vi "main battery tester vi22.vi"() -> ()   [LabVIEW 2019]
uses:
  Test_State_Enum.ctl
panel:
  out "system fault":bool
  in  "Start":bool
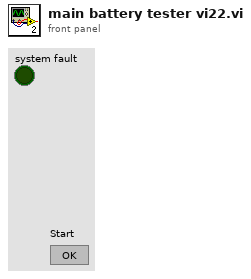
[diagram p1: front panel]
types:
  T1 = enum16{"open", "open or create", "create or replace", "create", "open (read-only)"}
  T2 = typedef "Test_State_Enum.ctl" = enum16{"INIT", "IDLE", "CHARGE _CC", "CHARGE _CV", "REST", "DISCHARGE_DC", "Fault", "Stop"}
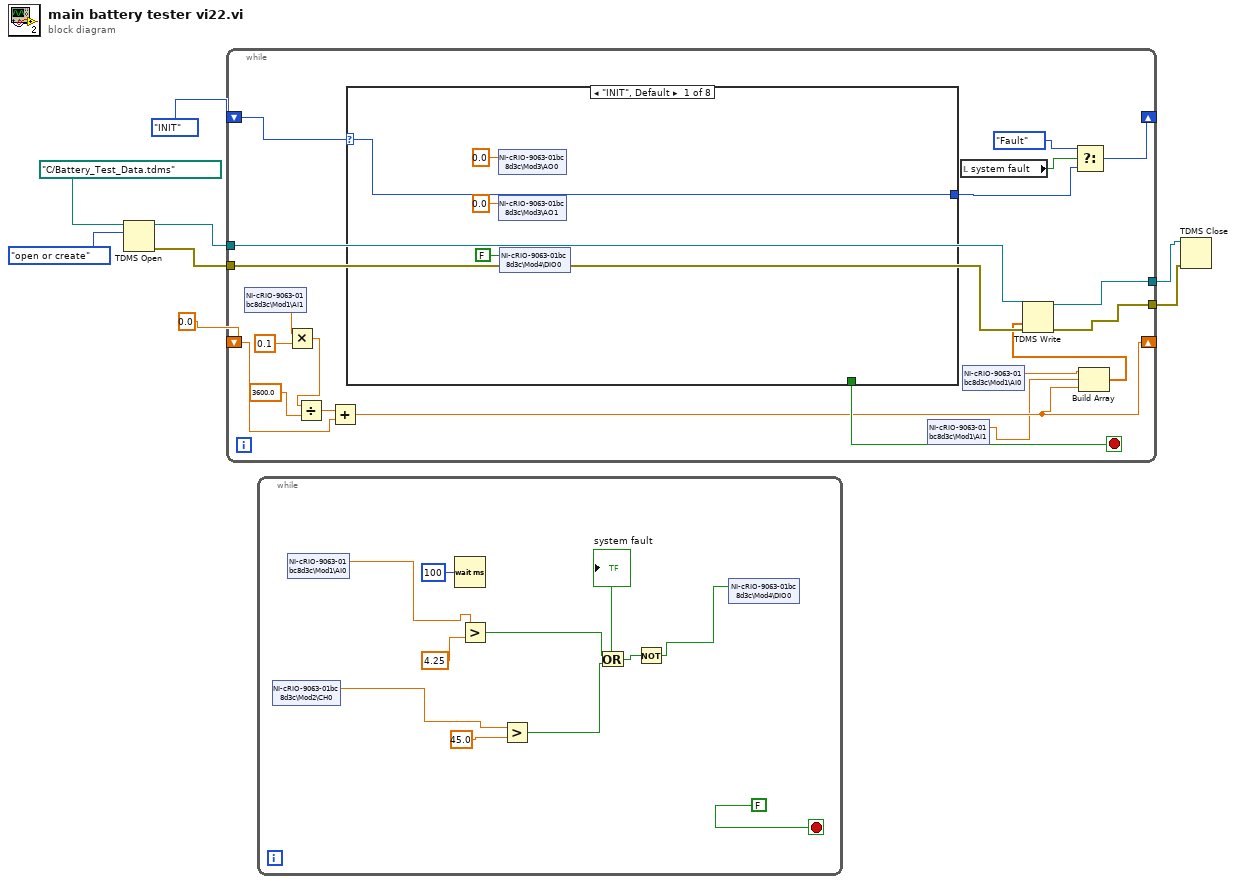
[diagram p0: block diagram]
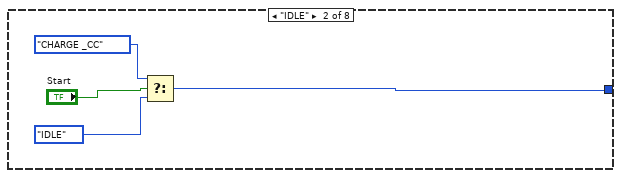
[diagram p2: hidden frame]
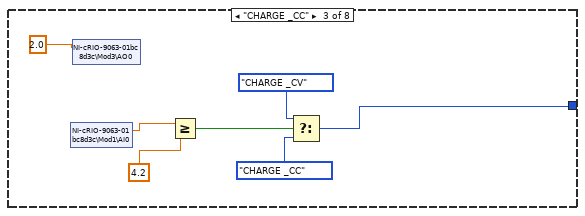
[diagram p3: hidden frame]
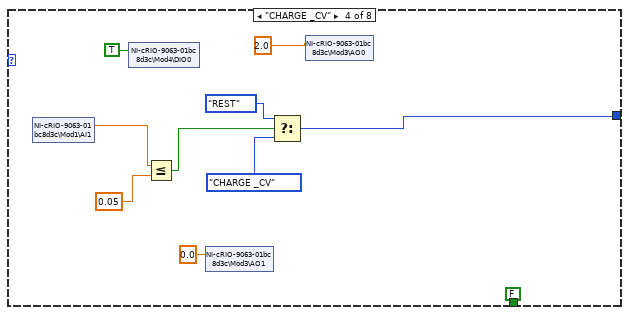
[diagram p4: hidden frame]
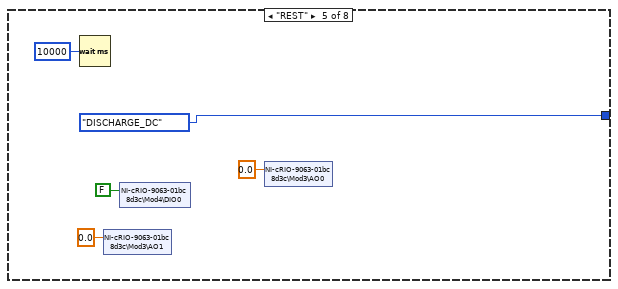
[diagram p5: hidden frame]
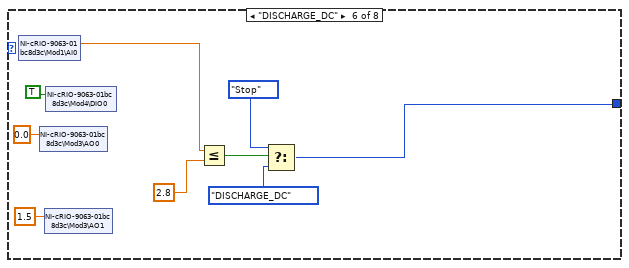
[diagram p6: hidden frame]
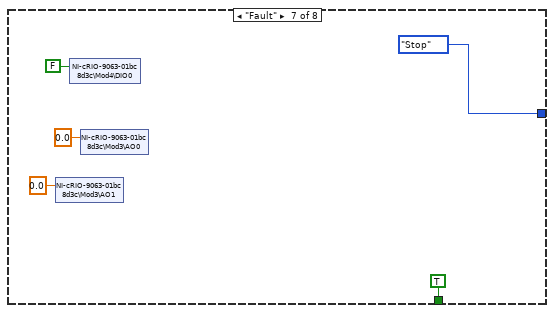
[diagram p7: hidden frame]
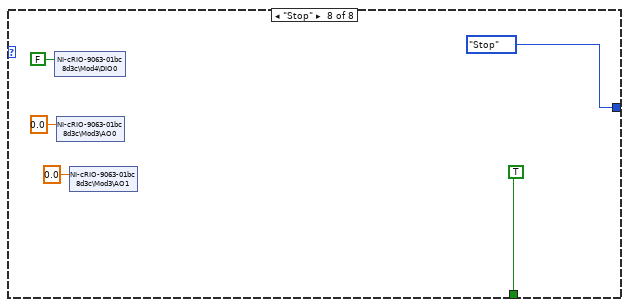
[diagram p8: hidden frame]
diagram:
  n1 = TDMS Open(10:T1."open or create" ("operation (0:open)"), 11:path "C:/Battery_Test_Data.tdms" ("file path")) -> (0:w5:errorcluster, 3:w6:refnum<k34>)  [unwired: 5 in]
  n2 = while {
    shift-right: [w23] -> _
    shift-left: Test_State_Enum."INIT" ("Enum") -> [w28]
    tunnel: w6 -> [w18]
    tunnel: w5 -> [w17]
    shift-right: [w16] -> _
    shift-left: 0.0 -> [w11]
    tunnel: [w15] -> w3
    tunnel: [w14] -> w2
    stop <- w27 stop-if-true
    n3 = shared-variable "NI-cRIO-9063-01bc8d3c\\Mod1\\AI1"() -> (w12:dbl)  [unwired: 1 in, 1 out]
    n4 = Multiply(x=w12, y=0.1) -> (x*y=w21:dbl)
    n5 = Divide(x=w21, y=3600.0) -> (x/y=w19:dbl)
    n6 = Add(x=w19, y=w11) -> (x+y=w16:dbl)
    n7 = case shown="\"INIT\", Default" w28 {
      selector: w28 -> [w29 _ _ _ _ _ _ _]
      tunnel: [w29 w34 w42 w49 Test_State_Enum."DISCHARGE_DC" ("Enum") w63 Test_State_Enum."Stop" ("Enum") Test_State_Enum."Stop" ("Enum")] -> w24
      tunnel: [_ _ _ FALSE ("stop") _ _ TRUE ("stop") TRUE ("stop")] -> w27
      frame "INIT", Default {
        n8 = shared-variable "NI-cRIO-9063-01bc8d3c\\Mod3\\AO0"(0.0 ("AO0")) -> ()  [unwired: 1 in, 1 out]
        n9 = shared-variable "NI-cRIO-9063-01bc8d3c\\Mod3\\AO1"(0.0 ("AO1")) -> ()  [unwired: 1 in, 1 out]
        n10 = shared-variable "NI-cRIO-9063-01bc8d3c\\Mod4\\DIO0"(FALSE ("DIO0")) -> ()  [unwired: 1 in, 1 out]
      }
      frame "IDLE" {
        n11 = Select(t=Test_State_Enum."CHARGE _CC" ("Enum"), s="Start", f=Test_State_Enum."IDLE" ("Enum")) -> (s? t:f=w34:T2)
      }
      frame "CHARGE _CC" {
        n12 = shared-variable "NI-cRIO-9063-01bc8d3c\\Mod1\\AI0"() -> (w38:dbl)  [unwired: 1 in, 1 out]
        n13 = shared-variable "NI-cRIO-9063-01bc8d3c\\Mod3\\AO0"(2.0 ("AO0")) -> ()  [unwired: 1 in, 1 out]
        n14 = Greater Or Equal?(x=w38, y=4.2) -> (x >= y?=w39:bool)
        n15 = Select(t=Test_State_Enum."CHARGE _CV" ("Enum"), s=w39, f=Test_State_Enum."CHARGE _CC" ("Enum")) -> (s? t:f=w42:T2)
      }
      frame "CHARGE _CV" {
        n16 = shared-variable "NI-cRIO-9063-01bc8d3c\\Mod1\\AI1"() -> (w46:dbl)  [unwired: 1 in, 1 out]
        n17 = shared-variable "NI-cRIO-9063-01bc8d3c\\Mod4\\DIO0"(TRUE ("DIO0")) -> ()  [unwired: 1 in, 1 out]
        n18 = Less Or Equal?(x=w46, y=0.05) -> (x <= y?=w50:bool)
        n19 = shared-variable "NI-cRIO-9063-01bc8d3c\\Mod3\\AO1"(0.0 ("AO1")) -> ()  [unwired: 1 in, 1 out]
        n20 = Select(t=Test_State_Enum."REST" ("Enum"), s=w50, f=Test_State_Enum."CHARGE _CV" ("Enum")) -> (s? t:f=w49:T2)
        n21 = shared-variable "NI-cRIO-9063-01bc8d3c\\Mod3\\AO0"(2.0 ("AO0")) -> ()  [unwired: 1 in, 1 out]
      }
      frame "REST" {
        n22 = Wait (ms)(milliseconds to wait=u32 10000) -> ()  [unwired: 1 out]
        n23 = shared-variable "NI-cRIO-9063-01bc8d3c\\Mod3\\AO1"(0.0 ("AO1")) -> ()  [unwired: 1 in, 1 out]
        n24 = shared-variable "NI-cRIO-9063-01bc8d3c\\Mod4\\DIO0"(FALSE ("DIO0")) -> ()  [unwired: 1 in, 1 out]
        n25 = shared-variable "NI-cRIO-9063-01bc8d3c\\Mod3\\AO0"(0.0 ("AO0")) -> ()  [unwired: 1 in, 1 out]
      }
      frame "DISCHARGE_DC" {
        n26 = shared-variable "NI-cRIO-9063-01bc8d3c\\Mod1\\AI0"() -> (w59:dbl)  [unwired: 1 in, 1 out]
        n27 = shared-variable "NI-cRIO-9063-01bc8d3c\\Mod3\\AO0"(0.0 ("AO0")) -> ()  [unwired: 1 in, 1 out]
        n28 = shared-variable "NI-cRIO-9063-01bc8d3c\\Mod3\\AO1"(1.5 ("AO1")) -> ()  [unwired: 1 in, 1 out]
        n29 = shared-variable "NI-cRIO-9063-01bc8d3c\\Mod4\\DIO0"(TRUE ("DIO0")) -> ()  [unwired: 1 in, 1 out]
        n30 = Less Or Equal?(x=w59, y=2.8) -> (x <= y?=w66:bool)
        n31 = Select(t=Test_State_Enum."Stop" ("Enum"), s=w66, f=Test_State_Enum."DISCHARGE_DC" ("Enum")) -> (s? t:f=w63:T2)
      }
      frame "Fault" {
        n32 = shared-variable "NI-cRIO-9063-01bc8d3c\\Mod3\\AO1"(0.0 ("AO1")) -> ()  [unwired: 1 in, 1 out]
        n33 = shared-variable "NI-cRIO-9063-01bc8d3c\\Mod4\\DIO0"(FALSE ("DIO0")) -> ()  [unwired: 1 in, 1 out]
        n34 = shared-variable "NI-cRIO-9063-01bc8d3c\\Mod3\\AO0"(0.0 ("AO0")) -> ()  [unwired: 1 in, 1 out]
      }
      frame "Stop" {
        n35 = shared-variable "NI-cRIO-9063-01bc8d3c\\Mod4\\DIO0"(FALSE ("DIO0")) -> ()  [unwired: 1 in, 1 out]
        n36 = shared-variable "NI-cRIO-9063-01bc8d3c\\Mod3\\AO0"(0.0 ("AO0")) -> ()  [unwired: 1 in, 1 out]
        n37 = shared-variable "NI-cRIO-9063-01bc8d3c\\Mod3\\AO1"(0.0 ("AO1")) -> ()  [unwired: 1 in, 1 out]
      }
    }
    n38 = shared-variable "NI-cRIO-9063-01bc8d3c\\Mod1\\AI1"() -> (w9:dbl)  [unwired: 1 in, 1 out]
    n39 = local read "system fault"() -> (w25:bool)
    n40 = shared-variable "NI-cRIO-9063-01bc8d3c\\Mod1\\AI0"() -> (w10:dbl)  [unwired: 1 in, 1 out]
    n41 = Select(t=Test_State_Enum."Fault", s=w25, f=w24) -> (s? t:f=w23:T2)
    n42 = Build Array(w10, w9, w16) -> (w13:dbl[])
    n43 = TDMS Write(0:w18, 9:w13, 11:w17) -> (4:w15:refnum<k34>, 15:w14:errorcluster)  [unwired: 3 in, 2 out]
  }
  n44 = while {
    stop <- FALSE stop-if-true
    n45 = shared-variable "NI-cRIO-9063-01bc8d3c\\Mod2\\CH0"() -> (w80:dbl)  [unwired: 1 in, 1 out]
    n46 = shared-variable "NI-cRIO-9063-01bc8d3c\\Mod1\\AI0"() -> (w81:dbl)  [unwired: 1 in, 1 out]
    n47 = Wait (ms)(milliseconds to wait=u32 100) -> ()  [unwired: 1 out]
    n48 = Greater?(x=w81, y=4.25) -> (0:w84:bool)
    n49 = Greater?(x=w80, y=45.0) -> (0:w83:bool)
    n50 = Or(x=w84, y=w83) -> (x .or. y?=w82:bool)
    "system fault" <- w82
    n51 = Not(x=w82) -> (.not. x?=w79:bool)
    n52 = shared-variable "NI-cRIO-9063-01bc8d3c\\Mod4\\DIO0"(w79) -> ()  [unwired: 1 in, 1 out]
  }
  n53 = TDMS Close(8:w2, 11:w3) -> ()  [unwired: 2 out]
